vi "BaseProvider_IniFileSettings.vi"(1 "IniFileSettings":T1, 5 "error in (no error)":errorcluster, 6 "Action":enum16{"Read", "Load", "Save"}(ring)) -> (15 "IniFileSettings":T1, 19 "error out":errorcluster)   [LabVIEW 2020]
uses:
  <resource>/Framework/Providers/Open_GDS/ClassProviders/Provider_BaseClassInterface/BaseProvider_SubVIs/BaseProvider_IniFileSettings.ctl
  <resource>/Framework/Providers/Open_GDS/ClassProviders/Provider_BaseClassInterface/BaseProvider_SubVIs/BaseProvider_FileNamingOption.ctl
  <vilib>/Utility/config.llb/Read Key (String).vi
  <vilib>/Utility/config.llb/Write Key (String).vi
  <vilib>/Utility/config.llb/NI_LVConfig.lvlib
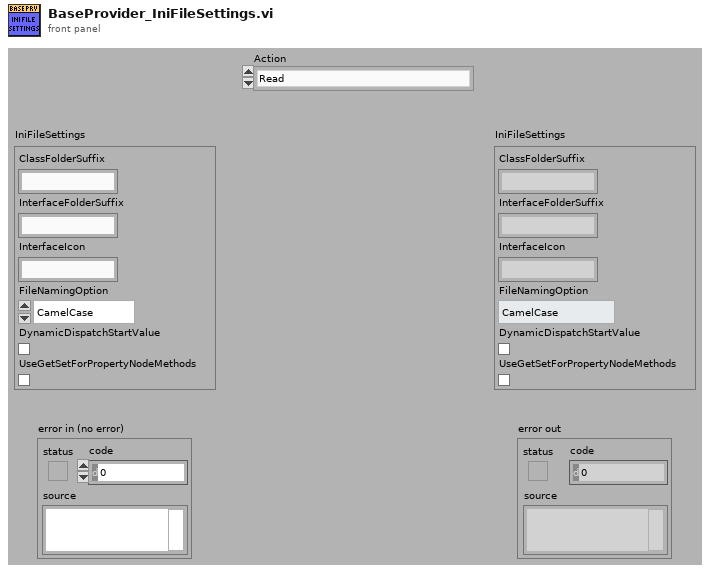
[diagram p1: front panel]
types:
  T1 = typedef "BaseProvider_IniFileSettings.ctl" = cluster{"ClassFolderSuffix":string, "InterfaceFolderSuffix":string, "InterfaceIcon":string, "FileNamingOption":T2, "DynamicDispatchStartValue":bool, "UseGetSetForPropertyNodeMethods":bool}
  T2 = typedef "BaseProvider_FileNamingOption.ctl" = enum16{"CamelCase", "Space", "Underscore"}
  T3 = typedef "NI_LVConfig.lvlib/Config Data RefNum.ctl" = refnum<k1>
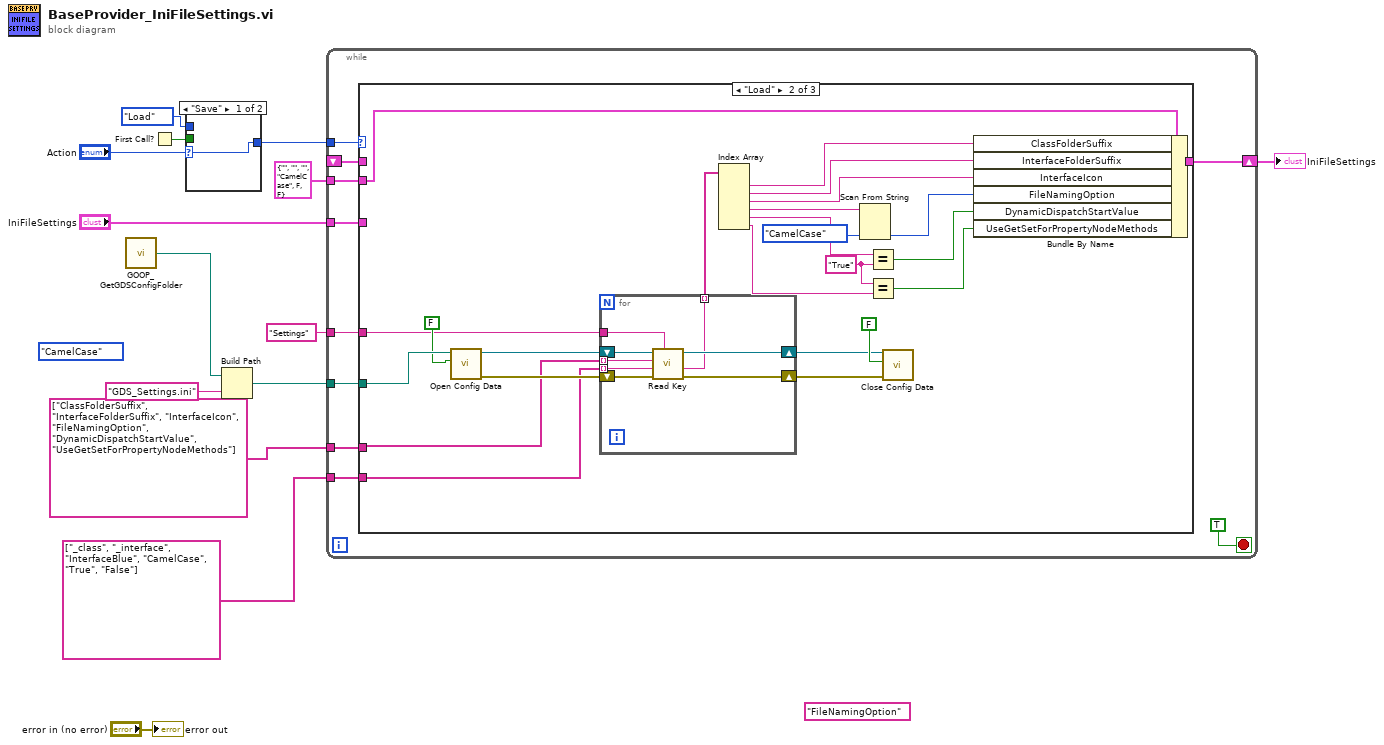
[diagram p0: block diagram]
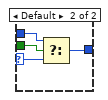
[diagram p2: hidden frame]
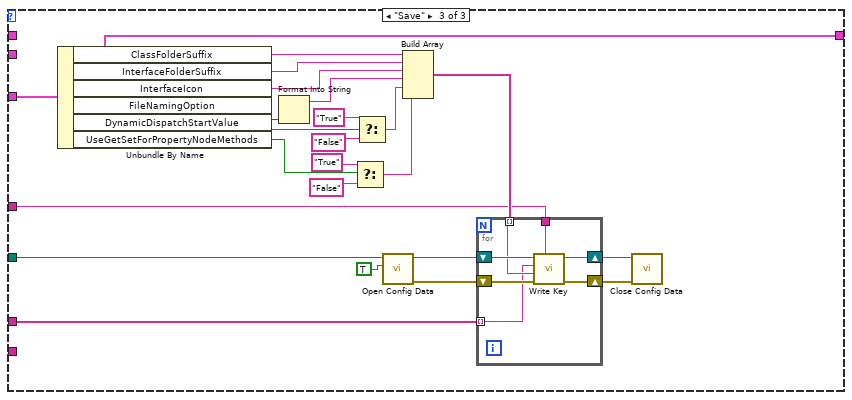
[diagram p4: hidden frame]
diagram:
  (unwired) BaseProvider_FileNamingOption."CamelCase" ("input 1")
  (unwired) "FileNamingOption" ("key")
  n1 = call <resource>:"GOOP_GetGDSConfigFolder.vi"() -> ("GDSFolderPath"=w13:path)
  n2 = First Call?() -> (First Call?: T/F=w10:bool)
  n3 = case shown="\"Save\"" "Action" {
    selector: "Action" -> [w15 w16]
    tunnel: w10 -> [_ w19]
    tunnel: [w15 w18] -> w9
    tunnel: enum16{"Read", "Load", "Save"}."Load" ("t") -> [_ w17]
    frame "Save" {
    }
    frame Default {
      n4 = Select(t=w17, s=w19, f=w16) -> (s? t:f=w18:enum16{"Read", "Load", "Save"})
    }
  }
  n5 = Build Path(base path=w13, name or relative path="GDS_Settings.ini") -> (appended path=w12:path)
  n6 = while {
    tunnel: w9 -> [w29]
    tunnel: w12 -> [w28]
    shift-right: [w26] -> w11
    shift-left: _ -> [w25]
    tunnel: "IniFileSettings" -> [w24]
    tunnel: T1 {"ClassFolderSuffix"="", "InterfaceFolderSuffix"="", "InterfaceIcon"="", "FileNamingOption"=enum."CamelCase", "DynamicDispatchStartValue"=FALSE, "UseGetSetForPropertyNodeMethods"=FALSE} ("IniFileSettings") -> [w23]
    tunnel: string[] ["ClassFolderSuffix", "InterfaceFolderSuffix", "InterfaceIcon", "FileNamingOption", "DynamicDispatchStartValue", "UseGetSetForPropertyNodeMethods"] -> [w22]
    tunnel: "Settings" ("section") -> [w21]
    tunnel: string[] ["_class", "_interface", "InterfaceBlue", "CamelCase", "True", "False"] -> [w20]
    stop <- TRUE stop-if-true
    n7 = case shown="\"Load\"" w29 {
      tunnel: w28 -> [_ w54 w84]
      tunnel: [w30 w49 w72] -> w26
      tunnel: w25 -> [w30 _ _]
      tunnel: w24 -> [_ _ w72]
      tunnel: w23 -> [_ w50 _]
      tunnel: w22 -> [_ w46 w73]
      tunnel: w21 -> [_ w47 w71]
      tunnel: w20 -> [_ w45 _]
      frame "Read", Default {
      }
      frame "Load" {
        w32 = "True" ("y")
        n8 = call <vilib>:"Open Config Data.vi"("create file if necessary (T)"=FALSE, "configuration file path"=w54) -> ("error out"=w52:errorcluster, "refnum"=w53:T3)  [unwired: 7 in, 1 out]
        n9 = for {
          tunnel: w47 -> [w60]
          tunnel: w46 -> [w59] mode=indexing
          tunnel: w45 -> [w58] mode=indexing
          shift-right: [w57] -> w44
          shift-left: w53 -> [w62]
          shift-right: [w56] -> w43
          shift-left: w52 -> [w61]
          tunnel: [w55] -> w42 mode=indexing
          n10 = call-poly <vilib>:"Read Key.vi"("section"=w60, "error in (no error)"=w61, "default value"=w58, "key"=w59, "refnum"=w62) -> ("error out"=w56:errorcluster, "value"=w55:string, "refnum out"=w57:T3)  [unwired: 3 in, 1 out]
        }
        n11 = Index Array(array=w42) -> (element #1=w36:string, element #2=w37:string, element #3=w38:string, element #4=w41:string, element #5=w35:string, element #6=w33:string)  [unwired: 6 in]
        n12 = Scan From String(input string=w41, default 1=BaseProvider_FileNamingOption."CamelCase" ("input 1")) -> (output 1=w39:T2)  [unwired: 3 in, 3 out]
        n13 = Equal?(x=w35, y=w32) -> (x = y?=w34:bool)
        n14 = Equal?(x=w32, y=w33) -> (x = y?=w31:bool)
        n15 = call <vilib>:"Close Config Data.vi"("error in (no error)"=w43, "write file if changed (T)"=FALSE, "refnum"=w44) -> ()  [unwired: 7 in, 2 out]
        n16 = Bundle By Name(cluster=w50, "ClassFolderSuffix"=w36, "InterfaceFolderSuffix"=w37, "InterfaceIcon"=w38, "FileNamingOption"=w39, "DynamicDispatchStartValue"=w34, "UseGetSetForPropertyNodeMethods"=w31) -> (w49:T1)
      }
      frame "Save" {
        n17 = Unbundle By Name(w72) -> ("ClassFolderSuffix"=w83:string, "InterfaceFolderSuffix"=w82:string, "InterfaceIcon"=w81:string, "FileNamingOption"=w79:T2, "DynamicDispatchStartValue"=w70:bool, "UseGetSetForPropertyNodeMethods"=w66:bool)
        n18 = Format Into String(w79) -> (resulting string=w80:string)  [unwired: 3 in, 1 out]
        n19 = Select(t="True" ("y"), s=w66, f="False" ("y")) -> (s? t:f=w63:string)
        n20 = Select(t="True" ("y"), s=w70, f="False" ("y")) -> (s? t:f=w69:string)
        n21 = call <vilib>:"Open Config Data.vi"("create file if necessary (T)"=TRUE, "configuration file path"=w84) -> ("error out"=w76:errorcluster, "refnum"=w78:T3)  [unwired: 7 in, 1 out]
        n22 = Build Array(w83, w82, w81, w80, w69, w63) -> (w74:string[])
        n23 = for {
          tunnel: w74 -> [w88] mode=indexing
          shift-right: [w91] -> w77
          shift-left: w78 -> [w92]
          shift-right: [w89] -> w75
          shift-left: w76 -> [w90]
          tunnel: w73 -> [w87] mode=indexing
          tunnel: w71 -> [w86]
          n24 = call-poly <vilib>:"Write Key.vi"("section"=w86, "error in (no error)"=w90, "value"=w88, "key"=w87, "refnum"=w92) -> ("error out"=w89:errorcluster, "refnum out"=w91:T3)  [unwired: 4 in, 1 out]
        }
        n25 = call <vilib>:"Close Config Data.vi"("error in (no error)"=w75, "refnum"=w77) -> ()  [unwired: 8 in, 2 out]
      }
    }
  }
  "IniFileSettings" <- w11
  "error out" <- "error in (no error)"
